vi "Generate Descriptor VI.vi"(8 "error in (no error)":errorcluster, 10 "Descriptor Strings":string[](array[string]), 11 "Library in":refnum<vi>) -> (0 "error out":errorcluster, 3 "Library out":refnum<vi>)   [LabVIEW 2019, in "gRPC Template Creation Utility.lvlib"]
uses:
  gRPC Template Creation Utility.lvlib
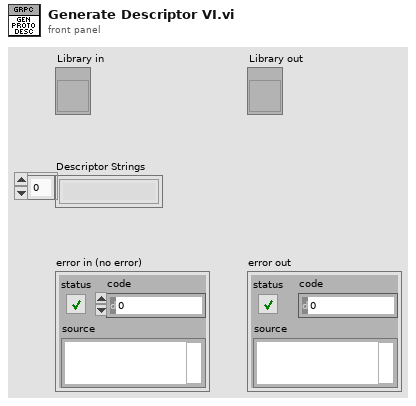
[diagram p1: front panel]
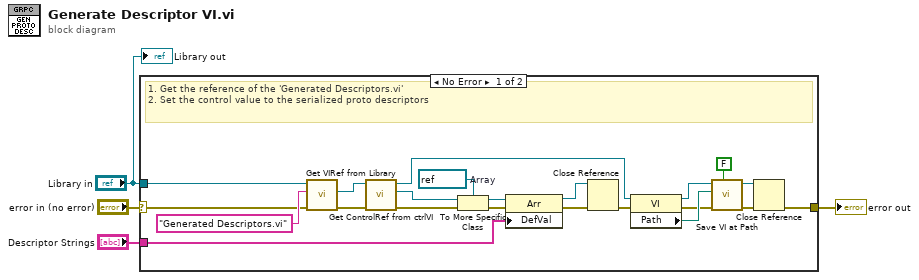
[diagram p0: block diagram]
diagram:
  n1 = case shown="No Error" "error in (no error)" {
    selector: "error in (no error)" -> [w19 w27]
    tunnel: [w9 w27] -> w4
    tunnel: "Library in" -> [w17 _]
    tunnel: "Descriptor Strings" -> [w18 _]
    frame No Error {
      w16 = refnum<vi> refnum  # Array
      # "1. Get the reference of the 'Generated Descriptors.vi'\n2. Set the control value to the serialized proto descriptors"
      n2 = call "Get VIRef from Library.vi"("error in (no error)"=w19, "Item Name"="Generated Descriptors.vi" ("Folder Name"), "Library"=w17) -> ("error out"=w14:errorcluster, "VIref out"=w15:refnum<vi>)  [unwired: 5 in, 2 out]
      n3 = call "Get ControlRef from ctrlVI.vi"("error in (no error)"=w14, "VI ref in"=w15) -> ("error out"=w12:errorcluster, "Control ref out"=w11:refnum<vi>, "VI ref out"=w13:refnum<vi>)  [unwired: 7 in]
      n4 = To More Specific Class(target class=w16, reference=w11, error in=w12) -> (specific class reference=w22:refnum<vi>, error out=w6:errorcluster)
      n5 = property class="Arr"(reference=w22, error in=w6, "DefVal"=w18) -> (reference out=w21:refnum<vi>, error out=w5:errorcluster)
      n6 = Close Reference(reference=w21, error in (no error)=w5) -> (error out=w8:errorcluster)
      n7 = property class="VI"(reference=w13, error in=w8) -> (reference out=w10:refnum<vi>, error out=w7:errorcluster, "Path"=w24:path)
      n8 = call "Save VI at Path.vi"("Override Existing? (T)"=FALSE, "error in (no error)"=w7, "Path"=w24, "VI in"=w10) -> ("error out"=w26:errorcluster, "VI out"=w25:refnum<vi>)  [unwired: 5 in, 1 out]
      n9 = Close Reference(reference=w25, error in (no error)=w26) -> (error out=w9:errorcluster)
    }
    frame Error {
    }
  }
  "error out" <- w4
  "Library out" <- "Library in"
